vi "PathPlanner_ConstraintsZone_New.vi"(9 "Constraints":T1, 10 "maxPosition":dbl, 11 "minPosition":dbl) -> (3 "ConstraintsZone":T2)   [LabVIEW 2019, in "PathPlanner24.lvlib"]
doc: "Create a new constraints zone\n\nInputs: \n -- MinPosition - double - Starting waypoint relative position of the zone\n -- MaxPosition - double - End waypoint relative position of the zone\n -- constraints - cluster - The constraints to apply within the zone\n\nOutputs:\n -- ConstraintsZone - cluster - data cluster with constraint"
uses:
  PathPlanner24.lvlib
  TypeDef/PathPlannerConstraintsZone.ctl
  TypeDef/PathPlannerPathConstraints.ctl
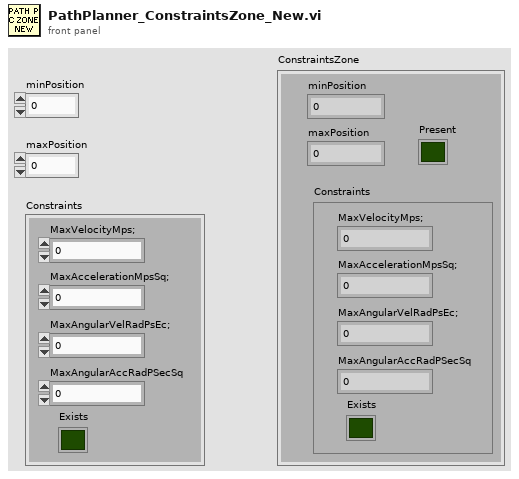
[diagram p1: front panel]
types:
  T1 = typedef "PathPlanner24.lvlib/PathPlannerPathConstraints.ctl" = cluster{"MaxVelocityMps;":dbl, "MaxAccelerationMpsSq;":dbl, "MaxAngularVelRadPsEc;":dbl, "MaxAngularAccRadPSecSq":dbl, "Exists":bool}
  T2 = typedef "PathPlanner24.lvlib/PathPlannerConstraintsZone.ctl" = cluster{"minPosition":dbl, "maxPosition":dbl, "Constraints":T1, "Present":bool}
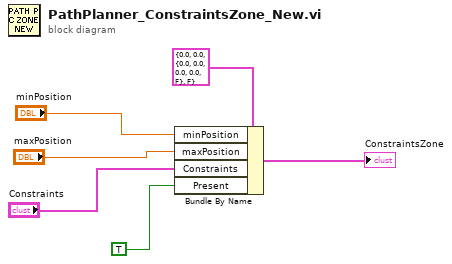
[diagram p0: block diagram]
diagram:
  n1 = Bundle By Name(cluster=T2 {"minPosition"=0.0, "maxPosition"=0.0, "Constraints"={"MaxVelocityMps;"=0.0, "MaxAccelerationMpsSq;"=0.0, "MaxAngularVelRadPsEc;"=0.0, "MaxAngularAccRadPSecSq"=0.0, "Exists"=FALSE}, "Present"=FALSE} ("ConstraintsZone"), "minPosition"="minPosition", "maxPosition"="maxPosition", "Constraints"="Constraints", "Present"=TRUE) -> (→"ConstraintsZone":T2)
